vi "Write Hardware Configuration.vi"(8 "error in":errorcluster, 10 "path":path, 11 "custom device":T1 format="%.0x") -> (0 "error out":errorcluster, 2 "path out":path, 3 "custom device out":T1 format="%.0x")   [LabVIEW 2020, in "Ballard ARINC 429 Hardware Configuration.lvlib"]
uses:
  Ballard ARINC 429 Hardware Configuration.lvlib
  <vilib>/NI VeriStand/Custom Device API/Custom Device Item Ref.ctl
  <vilib>/NI VeriStand/Custom Device API/Custom Device API.lvlib
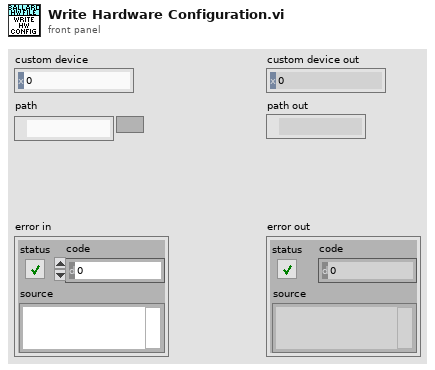
[diagram p1: front panel]
types:
  T1 = typedef "Custom Device API.lvlib/Custom Device Item Ref.ctl" = u64
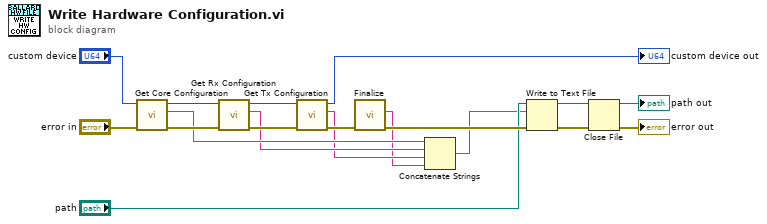
[diagram p0: block diagram]
diagram:
  n1 = call "Get Core Configuration.vi"("error in"="error in", "custom device"="custom device") -> ("error out"=w14:errorcluster, "configuration string"=w8:string, "custom device out"=w13:T1)  [unwired: 7 in]
  n2 = call "Get Rx Configuration.vi"("error in"=w14, "custom device"=w13) -> ("error out"=w12:errorcluster, "configuration string out"=w7:string, "custom device out"=w10:T1)  [unwired: 7 in]
  n3 = call "Get Tx Configuration.vi"("error in"=w12, "custom device"=w10) -> ("error out"=w11:errorcluster, "configuration string out"=w6:string, "custom device out"=→"custom device out":T1)  [unwired: 7 in]
  n4 = call "Finalize.vi"("error in"=w11) -> ("error out"=w17:errorcluster, "configuration string out"=w5:string)  [unwired: 9 in]
  n5 = Concatenate Strings(w8, w7, w6, w5) -> (w4:string)
  n6 = Write to Text File(file (use dialog)="path", text=w4, error in=w17) -> (refnum out=w2:refnum<file>, error out=w16:errorcluster)  [unwired: 1 in, 1 out]
  n7 = Close File(refnum=w2, error in=w16) -> (path=→"path out":path, error out=→"error out":errorcluster)
